vi "detect chassis.vi"(8 "error in":errorcluster, 11 "controller in":refnum<class "Controller.lvclass">) -> (0 "error out":errorcluster, 3 "controller out":refnum<class "Controller.lvclass">)   [LabVIEW 2014, in "SMI.lvlib" / "Controller.lvclass"]
uses:
  Controller.lvclass
  SysCfg Device/read system session.vi
  SysCfg Device/write system session.vi
  write local chassis.vi
  write remote chassis.vi
  Chassis/Chassis.lvclass
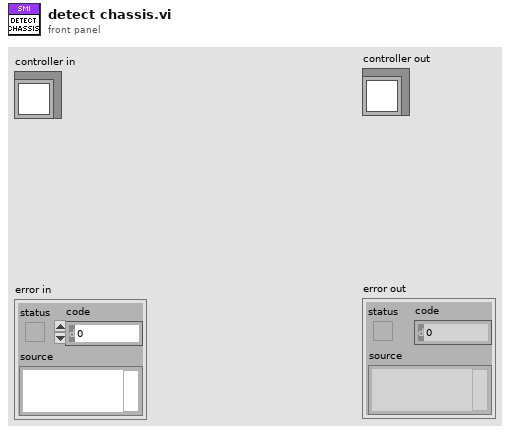
[diagram p1: front panel]
types:
  T1 = typedef "SMI.lvlib/Chassis.lvclass/chassis information.ctl" = cluster{"resource name":string, "vendor name":string, "product name":string, "product ID":u16, "serial number":string, "number of slots":i32, "device class":string}
  T2 = cluster{"local chassis":T1[], "remote chassis":T1[]}
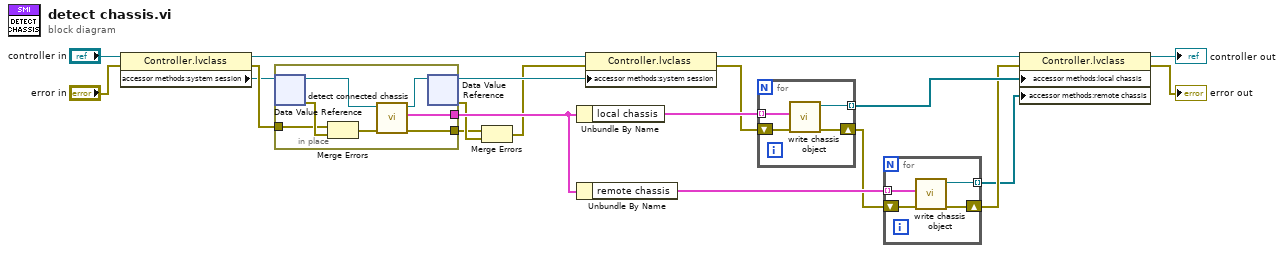
[diagram p0: block diagram]
diagram:
  n1 = property class="Controller.lvclass"(reference="controller in", error in="error in") -> (reference out=w18:refnum<class "Controller.lvclass">, error out=w20:errorcluster, "accessor methods:system session"=w11:refnum<data-value>)
  n2 = in-place {
    in-place-border: w20 -> [w22]
    in-place-border: [w27] -> w7
    in-place-border: [w26] -> w17
    n3 = in-place-dvr #1(w11) -> (w24:refnum<k21>, w23:errorcluster)
    n4 = Merge Errors(w22, w23) -> (w21:errorcluster)
    n5 = call "detect connected chassis.vi"("error in"=w21, "system session in"=w24) -> ("error out"=w27:errorcluster, "chassis"=w26:T2, "system session out"=w25:refnum<k21>)  [unwired: 7 in]
    n6 = in-place-dvr #1(w25) -> (w10:refnum<data-value>, w9:errorcluster)
  }
  n7 = Merge Errors(w7, w9) -> (w8:errorcluster)
  n8 = Unbundle By Name(w17) -> ("local chassis"=w15:T1[])
  n9 = Unbundle By Name(w17) -> ("remote chassis"=w16:T1[])
  n10 = property class="Controller.lvclass"(reference=w18, error in=w8, "accessor methods:system session"=w10) -> (reference out=w5:refnum<class "Controller.lvclass">, error out=w14:errorcluster)
  n11 = for {
    tunnel: w15 -> [w31] mode=indexing
    shift-right: [w29] -> w13
    shift-left: w14 -> [w30]
    tunnel: [w28] -> w6 mode=indexing
    n12 = call "write chassis object.vi"("error in"=w30, "chassis information"=w31) -> ("error out"=w29:errorcluster, "Chassis out"=w28:refnum<class "Chassis.lvclass">)  [unwired: 8 in]
  }
  n13 = for {
    tunnel: w16 -> [w35] mode=indexing
    shift-right: [w33] -> w4
    shift-left: w13 -> [w34]
    tunnel: [w32] -> w3 mode=indexing
    n14 = call "write chassis object.vi"("error in"=w34, "chassis information"=w35) -> ("error out"=w33:errorcluster, "Chassis out"=w32:refnum<class "Chassis.lvclass">)  [unwired: 8 in]
  }
  n15 = property class="Controller.lvclass"(reference=w5, error in=w4, "accessor methods:local chassis"=w6, "accessor methods:remote chassis"=w3) -> (reference out=→"controller out":refnum<class "Controller.lvclass">, error out=→"error out":errorcluster)
